vi "VIH HelpGen - Build - VIs.vi"(8 "error in":errorcluster, 9 "File paths":path[](array[path]), 10 "Items":T2, 11 "Project Tree":T1) -> (0 "error out":errorcluster, 2 "Items out":T2, 3 "dup Project Tree":T1)   [LabVIEW 2014]
doc: "::: VI Helpeks :::\nCopyright (c) 2000-2026 Konstantin Shifershteyn. All rights reserved."
uses:
  _VIH Project Manager.llb/VIH Project Tree Typedef - Tree Refnum.ctl
panel:
  # "VI Helpeks\nCopyright (c) 2012-2026 Konstantin Shifershteyn"
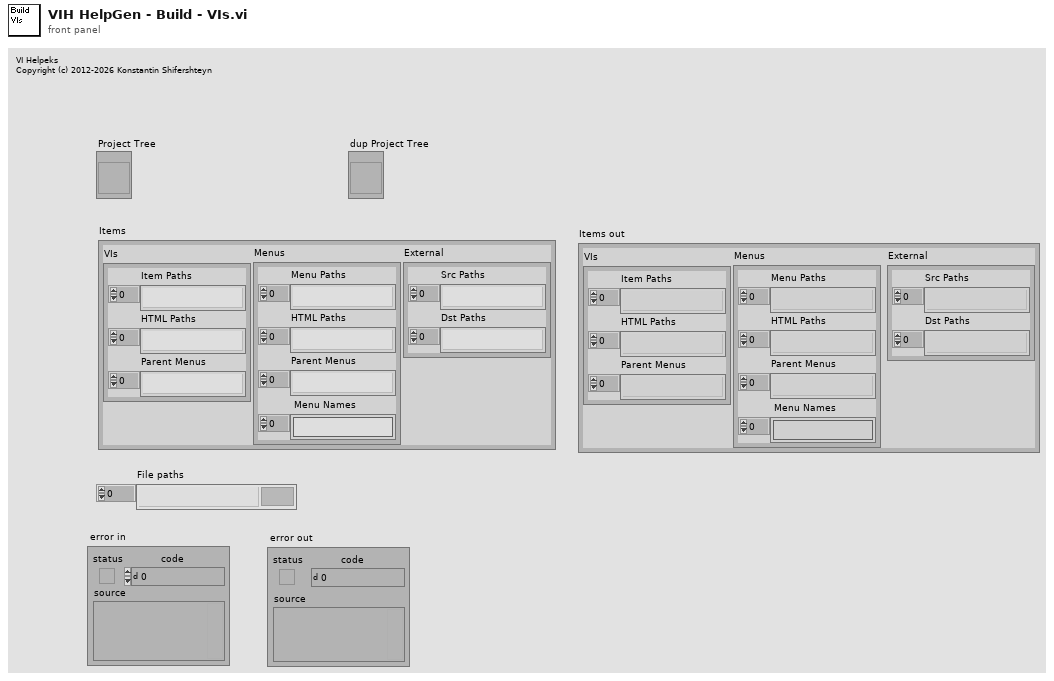
[diagram p1: front panel]
types:
  T1 = typedef "VIH Project Tree Typedef - Tree Refnum.ctl" = refnum<vi>
  T2 = cluster{"VIs":cluster{"Item Paths":path[], "HTML Paths":path[], "Parent Menus":path[]}, "Menus":cluster{"Menu Paths":path[], "HTML Paths":path[], "Parent Menus":path[], " Menu Names":string[]}, "External":cluster{"Src Paths":path[], "Dst Paths":path[]}}
  T3 = enum16{"nop", "Start", "Stop", "Run-prep", "Run-VI", "Run-Menu"}
  T4 = cluster{"Item Paths":path[], "HTML Paths":path[], "Parent Menus":path[]}
  T5 = cluster{"Menu Paths":path[], "HTML Paths":path[], "Parent Menus":path[], " Menu Names":string[]}
  T6 = typedef "VIH HelpGen Typedef - Palette - Item Type Enum.ctl" = enum32{"<Invalid>", "<unknown>", "VI", "Menu", "LV Func", "Express VI", "Poly VI", "CTL", "HTML"}
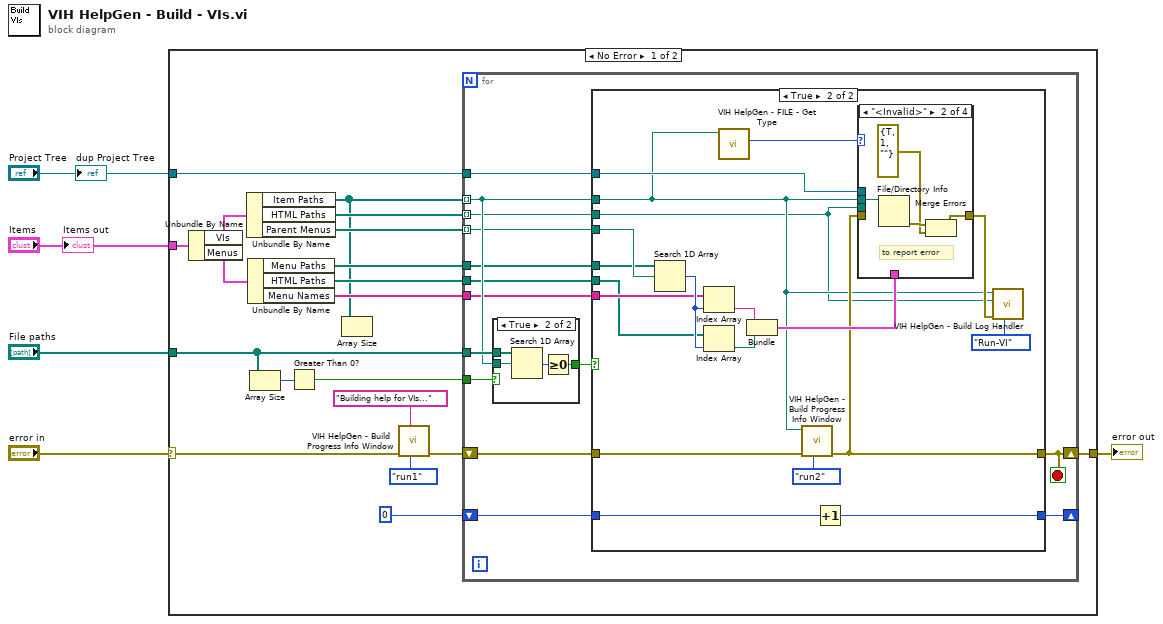
[diagram p0: block diagram]
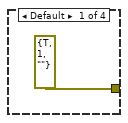
[diagram p3: hidden frame]
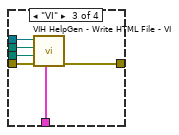
[diagram p4: hidden frame]
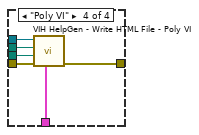
[diagram p5: hidden frame]
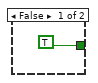
[diagram p6: hidden frame]
diagram:
  n1 = case shown="No Error" "error in" {
    selector: "error in" -> [w6 w82]
    tunnel: "File paths" -> [w24 _]
    tunnel: [w22 w82] -> w4
    tunnel: "Items" -> [w20 _]
    tunnel: "Project Tree" -> [w7 _]
    frame No Error {
      n2 = Unbundle By Name(w20) -> ("VIs"=w21:T4, "Menus"=w17:T5)
      n3 = Unbundle By Name(w21) -> ("Item Paths"=w8:path[], "HTML Paths"=w23:path[], "Parent Menus"=w19:path[])
      n4 = Unbundle By Name(w17) -> ("Menu Paths"=w18:path[], "HTML Paths"=w15:path[], "Menu Names"=w16:string[])
      n5 = Array Size(array=w24) -> (size(s)=w9:i32)
      n6 = Greater Than 0?(x=w9) -> (x > 0?=w10:bool)
      n7 = Array Size(array=w8) -> ()  [unwired: 1 out]
      n8 = call "VIH HelpGen - Build Progress Info Window.vi"("Mode (run1)"=enum16{"start", "stop", "run1", "run2"}."run1" ("Mode (run)"), "Message"="Building help for VIs...", "error in"=w6) -> ("error out"=w14:errorcluster)  [unwired: 8 in]
      n9 = for {
        tunnel: w10 -> [w38]
        tunnel: w24 -> [w37]
        tunnel: w8 -> [w35] mode=indexing
        tunnel: w23 -> [w34] mode=indexing
        shift-right: [w25] -> w22
        shift-left: w14 -> [w33]
        tunnel: w19 -> [w32] mode=indexing
        tunnel: w18 -> [w31]
        tunnel: w16 -> [w30]
        tunnel: w15 -> [w29]
        shift-right: [w27] -> _
        shift-left: 0 -> [w28]
        tunnel: w7 -> [w26]
        stop <- w25 stop-if-true
        n10 = case shown="True" w38 {
          tunnel: w37 -> [_ w81]
          tunnel: w35 -> [_ w80]
          tunnel: [TRUE w78] -> w36
          frame False {
          }
          frame True {
            n11 = Search 1D Array(1D array=w81, element=w80) -> (index of element=w79:i32)  [unwired: 1 in]
            n12 = Greater Or Equal To 0?(x=w79) -> (x >= 0?=w78:bool)
          }
        }
        n13 = case shown="True" w36 {
          tunnel: w35 -> [_ w43]
          tunnel: w34 -> [_ w41]
          tunnel: w33 -> [w40 w51]
          tunnel: [w40 w44] -> w25
          tunnel: w32 -> [_ w56]
          tunnel: w31 -> [_ w55]
          tunnel: w30 -> [_ w54]
          tunnel: w29 -> [_ w53]
          tunnel: w28 -> [w39 w50]
          tunnel: [w39 w49] -> w27
          tunnel: w26 -> [_ w47]
          frame False {
          }
          frame True {
            n14 = Search 1D Array(1D array=w55, element=w56) -> (index of element=w59:i32)  [unwired: 1 in]
            n15 = Index Array(array=w54, index=w59) -> (element=w58:string)
            n16 = Index Array(array=w53, index=w59) -> (element=w57:path)
            n17 = call "VIH HelpGen - FILE - Get Type.vi"("File Path"=w43) -> ("File Type"=w42:T6)  [unwired: 8 in, 2 out]
            n18 = Bundle("String"=w58, "Path"=w57) -> (w48:cluster{"String":string, "Path":path})  [unwired: 1 in]
            n19 = call "VIH HelpGen - Build Progress Info Window.vi"("Mode (run1)"=enum16{"start", "stop", "run1", "run2"}."run2" ("Mode (run)"), "error in"=w51, "Cur path"=w43) -> ("error out"=w44:errorcluster)  [unwired: 8 in]
            n20 = Increment(x=w50) -> (x+1=w49:i32)
            n21 = case shown="\"<Invalid>\"" w42 {
              tunnel: w48 -> [_ _ w70 w76]
              tunnel: w41 -> [_ _ w69 w75]
              tunnel: w47 -> [_ _ w68 w74]
              tunnel: w43 -> [_ w64 w67 w73]
              tunnel: [errorcluster {"status"=TRUE, "code"=1, "source"=""} ("error out") w61 w66 w72] -> w45
              tunnel: w44 -> [_ _ w65 w71]
              frame Default {
              }
              frame "<Invalid>" {
                # "to report error"
                n22 = File/Directory Info(path=w64) -> (error out=w63:errorcluster)  [unwired: 1 in, 6 out]
                n23 = Merge Errors(w63, errorcluster {"status"=TRUE, "code"=1, "source"=""} ("error out")) -> (w61:errorcluster)
              }
              frame "VI" {
                n24 = call "VIH HelpGen - Write HTML File - VI.vi"("Owning Palette"=w70, "error in"=w65, "HTML Path"=w69, "VI Path"=w67, "Project Tree"=w68) -> ("error out"=w66:errorcluster)  [unwired: 5 in, 1 out]
              }
              frame "Poly VI" {
                n25 = call "VIH HelpGen - Write HTML File - Poly VI.vi"("Owning Palette"=w76, "error in"=w71, "HTML Path"=w75, "VI Path"=w73, "Project Tree"=w74) -> ("error out"=w72:errorcluster)  [unwired: 5 in, 1 out]
              }
            }
            n26 = call "VIH HelpGen - Build Log Handler.vi"("cmd (nop)"=T3."Run-VI" ("cmd"), "error in"=w45, "Out File Path"=w41, "Src File Path"=w43) -> ()  [unwired: 3 in, 5 out]
          }
        }
      }
    }
    frame Error {
    }
  }
  "error out" <- w4
  "Items out" <- "Items"
  "dup Project Tree" <- "Project Tree"
